vi "HISW-Service.vi"(8 "error in (no error)":errorcluster, 11 "HISW in":refnum<class "HISW.lvclass">) -> (0 "error out":errorcluster, 3 "HISW out":refnum<class "HISW.lvclass">)   [LabVIEW 2020, in "Sgraph_lib_V1.lvlib" / "HISW.lvclass"]
doc: "HISW Service\n\nThis code snippet will receive all DAQ datagrams and pass it on to the AVPP"
uses:
  HISW.lvclass
  controls/typedef_PAQsample.ctl
  FAMM/controls/typedef_FAMM_Query.ctl
  FAMM/controls/typedef-functions.ctl
  controls/typedef-DAQ-datagram.ctl
  controls/typedef-Qtype.ctl
  FAMM/FAMM.lvclass
  HISW.lvclass/HISW.ctl
  Builds/Sgraph_lib_V1.lvlib
panel:
  in  "FAMM.lvclass":refnum<class "FAMM.lvclass">
  in  "DAQ-Queue":refnum<queue>
  out "# elements in queue":i32
  in  "FAMM-Queue":refnum<queue>
  out "PAQ-datagram":T1 {"data" format="%.2f"; "status" format="%08x"}
  out "iteration":i32
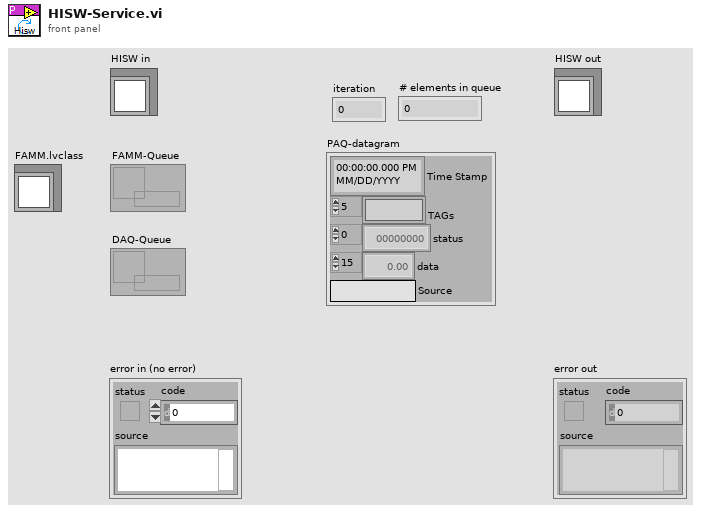
[diagram p1: front panel]
types:
  T1 = typedef "typedef_PAQsample.ctl" = cluster{"Time Stamp":timestamp, "TAGs":string[], "status":u32[], "data":dbl[], "Source":string}
  T2 = typedef "typedef-DAQ-datagram.ctl" = cluster{"Time Stamp":timestamp, "Source":string, "Data":variant, "Qtype":T3}
  T3 = typedef "typedef-Qtype.ctl" = enum16{"PAQ", "WAQ", "EAQ", "End-Service"}
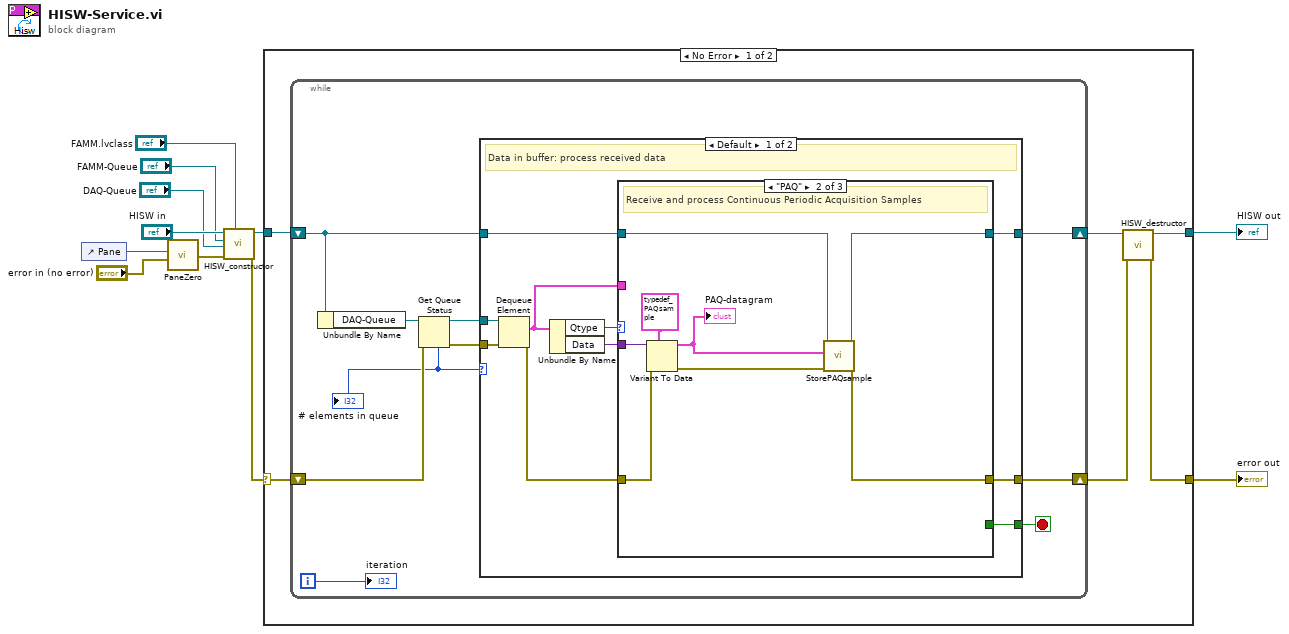
[diagram p0: block diagram]
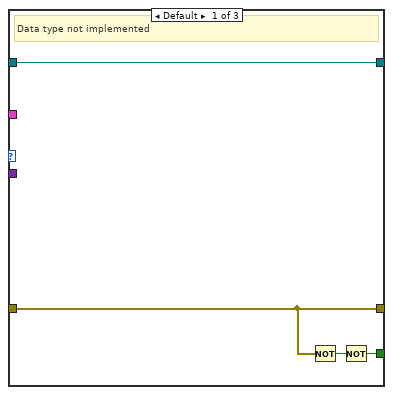
[diagram p2: hidden frame]
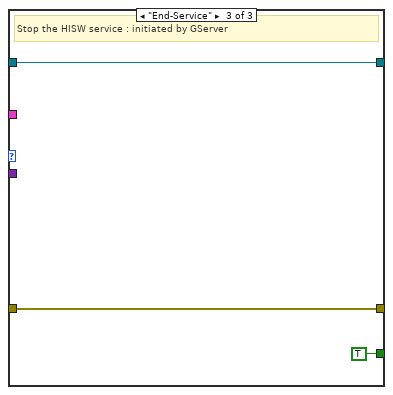
[diagram p3: hidden frame]
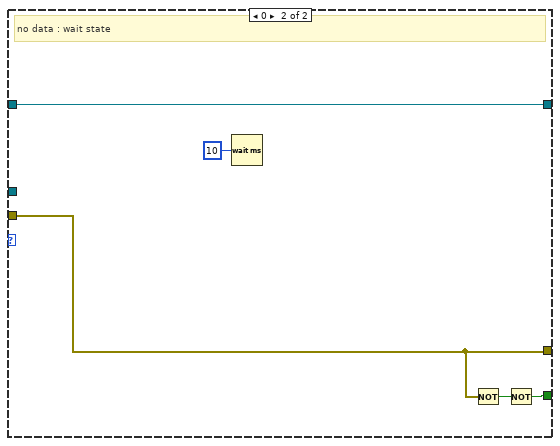
[diagram p4: hidden frame]
diagram:
  n1 = control-ref of="Pane"() -> (w4:refnum<vi>)
  n2 = call "PaneZero.vi"("error in (no error)"="error in (no error)", "Pane"=w4) -> ("error out"=w6:errorcluster)  [unwired: 9 in]
  n3 = call "HISW_constructor.vi"("FAMM.lvclass"="FAMM.lvclass", "error in (no error)"=w6, "DAQ-Queue"="DAQ-Queue", "FAMM-Queue"="FAMM-Queue", "HISW in"="HISW in") -> ("error out"=w7:errorcluster, "HISW out"=w8:refnum<class "HISW.lvclass">)  [unwired: 5 in]
  n4 = case shown="No Error" w7 {
    selector: w7 -> [w17 w59]
    tunnel: [w12 w59] -> w11
    tunnel: [w14 w58] -> w10
    tunnel: w8 -> [w16 w58]
    frame No Error {
      n5 = while {
        shift-right: [w23] -> w13
        shift-left: w17 -> [w26]
        shift-right: [w22] -> w15
        shift-left: w16 -> [w24]
        i -> [w19]
        stop <- w18 stop-if-true
        n6 = Unbundle By Name(w24) -> ("DAQ-Queue"=w27:refnum<queue>)
        n7 = Get Queue Status(queue=w27, error in (no error)=w26) -> (queue out=w21:refnum<queue>, error out=w20:errorcluster, # elements in queue=w25:i32)  [unwired: 1 in, 5 out]
        "# elements in queue" <- w25
        n8 = case shown="Default" w25 {
          tunnel: w24 -> [w33 w57]
          tunnel: [w31 w55] -> w23
          tunnel: [w32 w57] -> w22
          tunnel: w21 -> [w37 _]
          tunnel: w20 -> [w36 w55]
          tunnel: [w29 w53] -> w18
          frame Default {
            # "Data in buffer: process received data"
            n9 = Dequeue Element(queue=w37, error in (no error)=w36) -> (element=w30:T2, error out=w34:errorcluster)  [unwired: 1 in, 2 out]
            n10 = Unbundle By Name(w30) -> ("Qtype"=w35:T3, "Data"=w28:variant)
            n11 = case shown="\"PAQ\"" w35 {
              tunnel: w34 -> [w40 w48 w51]
              tunnel: w33 -> [w41 w45 w52]
              tunnel: [w41 w44 w52] -> w32
              tunnel: [w40 w42 w51] -> w31
              tunnel: w30 -> [_ _ _]
              tunnel: [w38 _ TRUE] -> w29
              tunnel: w28 -> [_ w49 _]
              frame Default {
                # "Data type not implemented"
                n12 = Not(x=w40) -> (.not. x?=w39:bool)
                n13 = Not(x=w39) -> (.not. x?=w38:bool)
              }
              frame "PAQ" {
                # "Receive and process Continuous Periodic Acquisition Samples"
                n14 = Variant To Data(error in=w48, type=T1 {"Time Stamp"=timestamp(0 s since 1904-01-01), "TAGs"=[], "status"=[], "data"=[], "Source"="DAQ"} ("PAQ IN"), Variant=w49) -> (data=w46:T1, error out=w43:errorcluster)
                "PAQ-datagram" <- w46
                n15 = call "StorePAQsample.vi"("error in (no error)"=w43, "PAQ IN"=w46, "HISW in"=w45) -> ("error out"=w42:errorcluster, "HISW out"=w44:refnum<class "HISW.lvclass">)  [unwired: 7 in]
              }
              frame "End-Service" {
                # "Stop the HISW service : initiated by GServer"
              }
            }
          }
          frame 0 {
            # "no data : wait state"
            n16 = Wait (ms)(milliseconds to wait=u32 10) -> ()  [unwired: 1 out]
            n17 = Not(x=w55) -> (.not. x?=w54:bool)
            n18 = Not(x=w54) -> (.not. x?=w53:bool)
          }
        }
        "iteration" <- w19
      }
      n19 = call "HISW_destructor.vi"("error in (no error)"=w13, "HISW in"=w15) -> ("error out"=w12:errorcluster, "HISW out"=w14:refnum<class "HISW.lvclass">)  [unwired: 8 in]
    }
    frame Error {
    }
  }
  "error out" <- w11
  "HISW out" <- w10
